vi "test.cfgTable.vi"() -> ()   [LabVIEW 2017]
uses:
  0ce3606b-4a8d-450a-b335-de3da5102bc9.vi
  baa86c02-3178-42a1-8f26-a93653cd2720.vi
  Configuration/ClusterCfgTable/Flatten Cluster To CfgTable(with DataName).vi
  Configuration/ClusterCfgTable/Parse CfgTable(with DataName).vi
panel:
  out "Cluster":cluster{dbl[unit], "DAQmx":tag}={123213.0, "DAQmx"=""}
  out "error out":errorcluster
  out "CfgTable Row":string[](array[string])
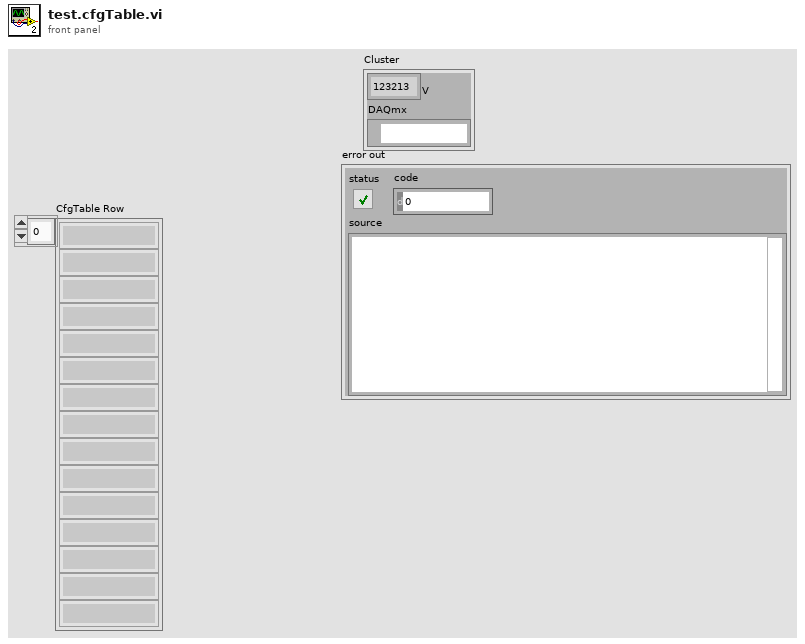
[diagram p1: front panel]
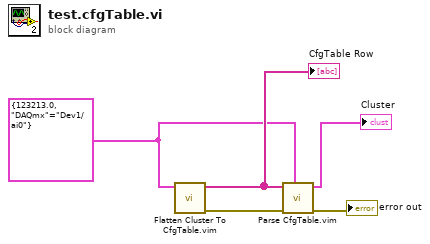
[diagram p0: block diagram]
diagram:
  w2 = cluster{dbl[unit], "DAQmx":tag} {123213.0, "DAQmx"="Dev1/ai0"}
  n1 = call "Flatten Cluster To CfgTable.vim"("Cluster Configuration Typedef"=w2) -> ("error out"=w4:errorcluster, "CfgTable Row"=w5:string[])  [unwired: 8 in, 1 out]
  "CfgTable Row" <- w5
  n2 = call "Parse CfgTable.vim"("Cluster Configuration Typedef"=w2, "error in (no error)"=w4, "CfgTable Row"=w5) -> ("error out"=→"error out":errorcluster, "Cluster Configuration Out"=→"Cluster":cluster{dbl[unit], "DAQmx":tag})  [unwired: 7 in]
